vi "Grade IO Test.vi"(8 "Data Map":T5(array[cluster]) {"OPC UA Data Type" items=["Boolean"=1, "SByte"=2, "Byte"=3, "Int16"=4, "UInt16"=5, "Int32"=6, "UInt32"=7, "Int64"=8, "UInt64"=9, "Float"=10, "Double"=11, "String"=12, "DateTime"=13, "ByteString"=15, "Array of Boolean"=101, "Array of SByte"=102, "Array of Byte"=103, "Array of Int16"=104, "Array of UInt16"=105, "Array of Int32"=106, "Array of UInt32"=107, "Array of Int64"=108, "Array of UInt64"=109, "Array of Float"=110, "Array of Double"=111, "Array of String"=112, "Array of DateTime"=113, "Array of ByteString"=115]}, 9 "Server Data":T1(array[cluster]), 10 "data table in":T2) -> (2 "Pass?":bool[](array[boolean]))   [LabVIEW 2014, in "OPC UA Client Tests.lvlib"]
doc: "Checks to see that the Server Data (data written using OPC UA Server API) matches what is in the module's data table. Input map is used to map data table items to server data items."
uses:
  OPC UA Client Tests.lvlib
  <vilib>/NI/Tag Bus/tag/Data Type.ctl
  module/configuration/OPC UA Data Type.ctl
  <vilib>/NI/Tag Bus/table/data table.ctl
  <vilib>/NI/Tag Bus/table/data polymorphs/read one/read Boolean.vi
  <vilib>/NI/Tag Bus/table/data polymorphs/read one/read I8.vi
  <vilib>/NI/Tag Bus/table/data polymorphs/read one/read U8.vi
  <vilib>/NI/Tag Bus/table/data polymorphs/read one/read I16.vi
  <vilib>/NI/Tag Bus/table/data polymorphs/read one/read U16.vi
  <vilib>/NI/Tag Bus/table/data polymorphs/read one/read I32.vi
  <vilib>/NI/Tag Bus/table/data polymorphs/read one/read U32.vi
  <vilib>/NI/Tag Bus/table/data polymorphs/read one/read I64.vi
  <vilib>/NI/Tag Bus/table/data polymorphs/read one/read U64.vi
  <vilib>/NI/Tag Bus/table/data polymorphs/read one/read Single.vi
  <vilib>/NI/Tag Bus/table/data polymorphs/read one/read Double.vi
  <vilib>/NI/Tag Bus/table/data polymorphs/read one/read String.vi
  <vilib>/NI/Tag Bus/table/data polymorphs/read one/read Array of Boolean.vi
  <vilib>/NI/Tag Bus/table/data polymorphs/read one/read Array of I8.vi
  <vilib>/NI/Tag Bus/table/data polymorphs/read one/read Array of U8.vi
  <vilib>/NI/Tag Bus/table/data polymorphs/read one/read Array of I16.vi
  <vilib>/NI/Tag Bus/table/data polymorphs/read one/read Array of U16.vi
  <vilib>/NI/Tag Bus/table/data polymorphs/read one/read Array of I32.vi
  <vilib>/NI/Tag Bus/table/data polymorphs/read one/read Array of U32.vi
  <vilib>/NI/Tag Bus/table/data polymorphs/read one/read Array of I64.vi
  <vilib>/NI/Tag Bus/table/data polymorphs/read one/read Array of U64.vi
  <vilib>/NI/Tag Bus/table/data polymorphs/read one/read Array of Single.vi
  <vilib>/NI/Tag Bus/table/data polymorphs/read one/read Array of Double.vi
  <vilib>/NI/Tag Bus/table/data polymorphs/read one/read Array of String.vi
  <vilib>/NI/Tag Bus/table/data table.lvlib
  module/execution/OPC UA Client runtime.lvclass
  <vilib>/NI/Tag Bus/tag/tag descriptor.lvclass
  module/configuration/OPC UA Client configuration.lvclass
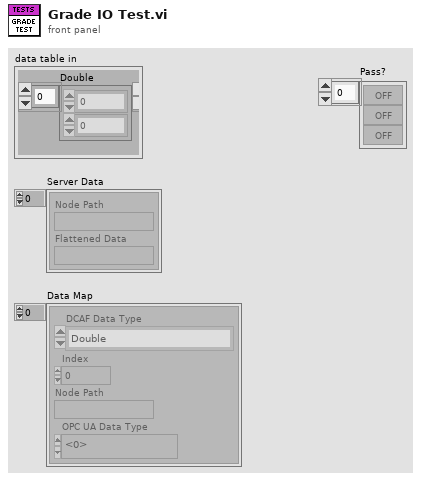
[diagram p1: front panel]
types:
  T1 = cluster{"Node Path":string, "Flattened Data":string}[]
  T2 = typedef "tag bus.lvlib/data table.lvlib/data table.ctl" = cluster{"Double":dbl[], "Single":sgl[], "I64":i64[], "I32":i32[], "I16":i16[], "I8":i8[], "U64":u64[], "U32":u32[], "U16":u16[], "U8":u8[], "Boolean":bool[], "String":string[], "Array of Double":cluster{"DBL Array":dbl[]}[], "Array of Single":cluster{"SGL Array":sgl[]}[], "Array of I64":cluster{"I64 Array":i64[]}[], "Array of I32":cluster{"I32 Array":i32[]}[], "Array of I16":cluster{"I16 Array":i16[]}[], "Array of I8":cluster{"I8 Array":i8[]}[], "Array of U64":cluster{"U64 Array":u64[]}[], "Array of U32":cluster{"U32 Array":u32[]}[], "Array of U16":cluster{"U16 Array":u16[]}[], "Array of U8":cluster{"U8 Array":u8[]}[], "Array of Boolean":cluster{"Boolean Array":bool[]}[], "Array of String":cluster{"String Array":string[]}[]}
  T3 = typedef "tag bus.lvlib/tag descriptor.lvclass/Data Type.ctl" = enum16{"Double", "Single", "I64", "I32", "I16", "I8", "U64", "U32", "U16", "U8", "Boolean", "String", "Array of Double", "Array of Single", "Array of I64", "Array of I32", "Array of I16", "Array of I8", "Array of U64", "Array of U32", "Array of U16", "Array of U8", "Array of Boolean", "Array of String"}
  T4 = typedef "OPC UA Client configuration.lvclass/OPC UA Data Type.ctl" = u16
  T5 = cluster{"DCAF Data Type":T3, "Index":i32, "Node Path":string, "OPC UA Data Type":T4}[]
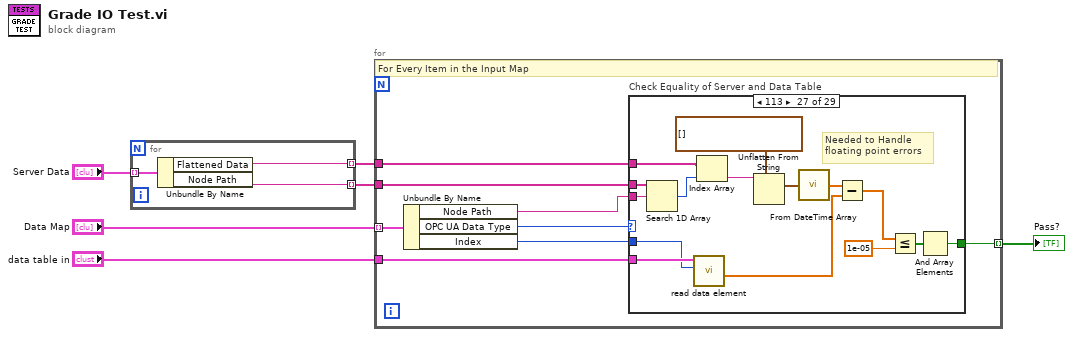
[diagram p0: block diagram]
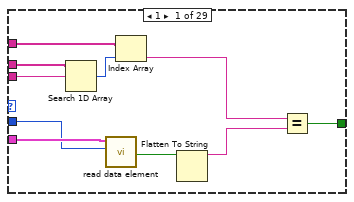
[diagram p2: hidden frame]
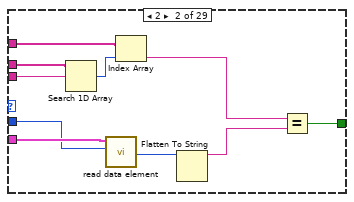
[diagram p3: hidden frame]
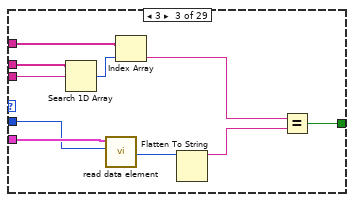
[diagram p4: hidden frame]
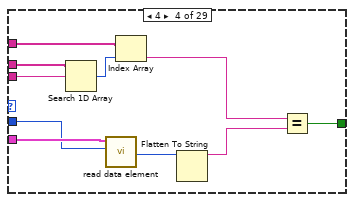
[diagram p5: hidden frame]
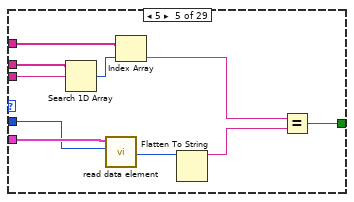
[diagram p6: hidden frame]
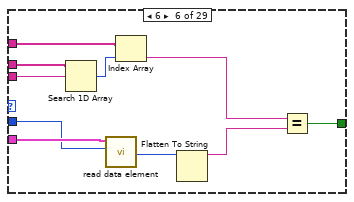
[diagram p7: hidden frame]
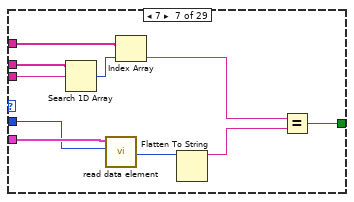
[diagram p8: hidden frame]
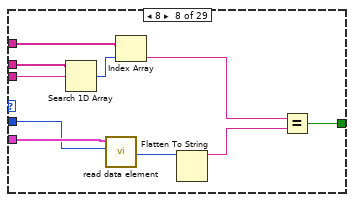
[diagram p9: hidden frame]
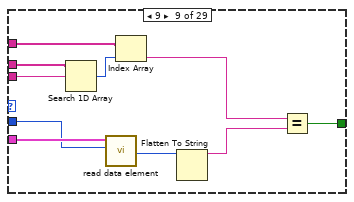
[diagram p10: hidden frame]
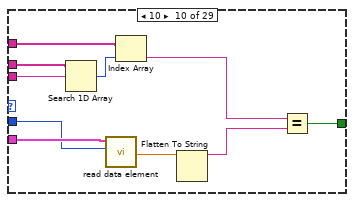
[diagram p11: hidden frame]
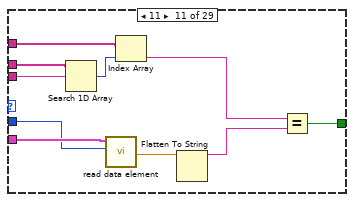
[diagram p12: hidden frame]
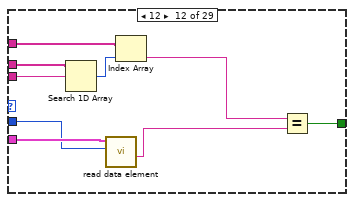
[diagram p13: hidden frame]
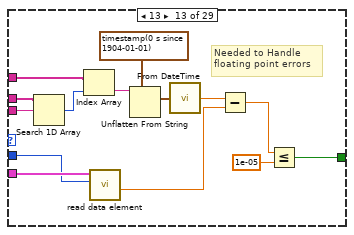
[diagram p14: hidden frame]
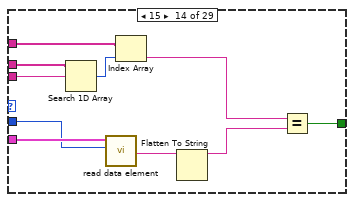
[diagram p15: hidden frame]
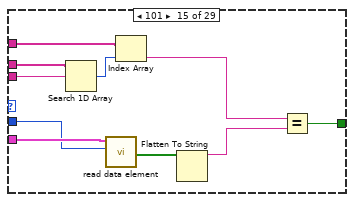
[diagram p16: hidden frame]
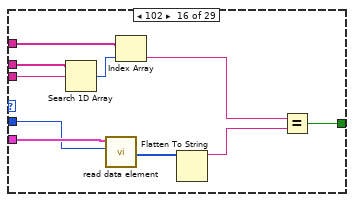
[diagram p17: hidden frame]
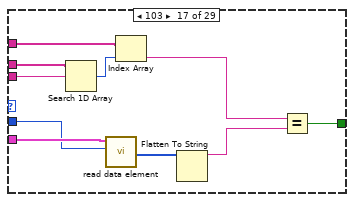
[diagram p18: hidden frame]
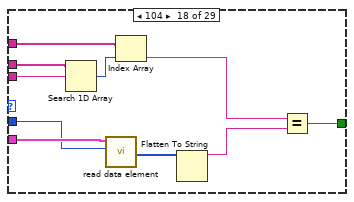
[diagram p19: hidden frame]
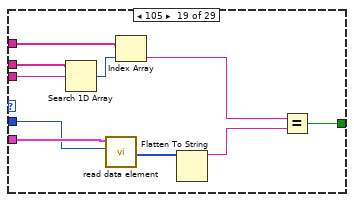
[diagram p20: hidden frame]
diagram:
  n1 = for {
    tunnel: "Server Data" -> [w9] mode=indexing
    tunnel: [w8] -> w3 mode=indexing
    tunnel: [w7] -> w2 mode=indexing
    n2 = Unbundle By Name(w9) -> ("Flattened Data"=w8:string, "Node Path"=w7:string)
  }
  n3 = for {
    tunnel: "Data Map" -> [w17] mode=indexing
    tunnel: "data table in" -> [w16]
    tunnel: w3 -> [w12]
    tunnel: w2 -> [w11]
    tunnel: [w10] -> w1 mode=indexing
    # "For Every Item in the Input Map"
    n4 = Unbundle By Name(w17) -> ("Node Path"=w14:string, "OPC UA Data Type"=w15:T4, "Index"=w13:i32)
    n5 = case "Check Equality of Server and Data Table" shown="113" w15 {
      tunnel: w16 -> [w23 w33 w43 w53 w63 w73 w83 w93 w103 w113 w123 w133 w149 w156 w166 w176 w186 w196 w206 w216 w226 w236 w246 w256 w266 w276 w294 w301 _]
      tunnel: w14 -> [w22 w32 w42 w52 w62 w72 w82 w92 w102 w112 w122 w132 w148 w155 w165 w175 w185 w195 w205 w215 w225 w235 w245 w255 w265 w275 w293 w300 _]
      tunnel: w13 -> [w21 w31 w41 w51 w61 w71 w81 w91 w101 w111 w121 w131 w147 w154 w164 w174 w184 w194 w204 w214 w224 w234 w244 w254 w264 w274 w292 w299 _]
      tunnel: w12 -> [w20 w30 w40 w50 w60 w70 w80 w90 w100 w110 w120 w130 w146 w153 w163 w173 w183 w193 w203 w213 w223 w233 w243 w253 w263 w273 w291 w298 _]
      tunnel: w11 -> [w19 w29 w39 w49 w59 w69 w79 w89 w99 w109 w119 w129 w145 w152 w162 w172 w182 w192 w202 w212 w222 w232 w242 w252 w262 w272 w290 w297 _]
      tunnel: [w18 w28 w38 w48 w58 w68 w78 w88 w98 w108 w118 w128 w138 w151 w161 w171 w181 w191 w201 w211 w221 w231 w241 w251 w261 w271 w281 w296 FALSE] -> w10
      frame 1 {
        n6 = Search 1D Array(1D array=w19, element=w22) -> (index of element=w25:i32)  [unwired: 1 in]
        n7 = call-poly <vilib>:"read data element.vi"("index"=w21, "data table in"=w23) -> ("value"=w24:bool)  [unwired: 8 in, 1 out]
        n8 = Index Array(array=w20, index=w25) -> (element=w27:string)
        n9 = Flatten To String(anything=w24) -> (data string=w26:string)  [unwired: 3 in, 2 out]
        n10 = Equal?(x=w27, y=w26) -> (x = y?=w18:bool)
      }
      frame 2 {
        n11 = Search 1D Array(1D array=w29, element=w32) -> (index of element=w35:i32)  [unwired: 1 in]
        n12 = call-poly <vilib>:"read data element.vi"("index"=w31, "data table in"=w33) -> ("value"=w34:i8)  [unwired: 8 in, 1 out]
        n13 = Index Array(array=w30, index=w35) -> (element=w37:string)
        n14 = Flatten To String(anything=w34) -> (data string=w36:string)  [unwired: 3 in, 2 out]
        n15 = Equal?(x=w37, y=w36) -> (x = y?=w28:bool)
      }
      frame 3 {
        n16 = Search 1D Array(1D array=w39, element=w42) -> (index of element=w45:i32)  [unwired: 1 in]
        n17 = call-poly <vilib>:"read data element.vi"("index"=w41, "data table in"=w43) -> ("value"=w44:u8)  [unwired: 8 in, 1 out]
        n18 = Index Array(array=w40, index=w45) -> (element=w47:string)
        n19 = Flatten To String(anything=w44) -> (data string=w46:string)  [unwired: 3 in, 2 out]
        n20 = Equal?(x=w47, y=w46) -> (x = y?=w38:bool)
      }
      frame 4 {
        n21 = Search 1D Array(1D array=w49, element=w52) -> (index of element=w55:i32)  [unwired: 1 in]
        n22 = call-poly <vilib>:"read data element.vi"("index"=w51, "data table in"=w53) -> ("value"=w54:i16)  [unwired: 8 in, 1 out]
        n23 = Index Array(array=w50, index=w55) -> (element=w57:string)
        n24 = Flatten To String(anything=w54) -> (data string=w56:string)  [unwired: 3 in, 2 out]
        n25 = Equal?(x=w57, y=w56) -> (x = y?=w48:bool)
      }
      frame 5 {
        n26 = Search 1D Array(1D array=w59, element=w62) -> (index of element=w65:i32)  [unwired: 1 in]
        n27 = call-poly <vilib>:"read data element.vi"("index"=w61, "data table in"=w63) -> ("value"=w64:u16)  [unwired: 8 in, 1 out]
        n28 = Index Array(array=w60, index=w65) -> (element=w67:string)
        n29 = Flatten To String(anything=w64) -> (data string=w66:string)  [unwired: 3 in, 2 out]
        n30 = Equal?(x=w67, y=w66) -> (x = y?=w58:bool)
      }
      frame 6 {
        n31 = Search 1D Array(1D array=w69, element=w72) -> (index of element=w75:i32)  [unwired: 1 in]
        n32 = call-poly <vilib>:"read data element.vi"("index"=w71, "data table in"=w73) -> ("value"=w74:i32)  [unwired: 8 in, 1 out]
        n33 = Index Array(array=w70, index=w75) -> (element=w77:string)
        n34 = Flatten To String(anything=w74) -> (data string=w76:string)  [unwired: 3 in, 2 out]
        n35 = Equal?(x=w77, y=w76) -> (x = y?=w68:bool)
      }
      frame 7 {
        n36 = Search 1D Array(1D array=w79, element=w82) -> (index of element=w85:i32)  [unwired: 1 in]
        n37 = call-poly <vilib>:"read data element.vi"("index"=w81, "data table in"=w83) -> ("value"=w84:u32)  [unwired: 8 in, 1 out]
        n38 = Index Array(array=w80, index=w85) -> (element=w87:string)
        n39 = Flatten To String(anything=w84) -> (data string=w86:string)  [unwired: 3 in, 2 out]
        n40 = Equal?(x=w87, y=w86) -> (x = y?=w78:bool)
      }
      frame 8 {
        n41 = Search 1D Array(1D array=w89, element=w92) -> (index of element=w95:i32)  [unwired: 1 in]
        n42 = call-poly <vilib>:"read data element.vi"("index"=w91, "data table in"=w93) -> ("value"=w94:i64)  [unwired: 8 in, 1 out]
        n43 = Index Array(array=w90, index=w95) -> (element=w97:string)
        n44 = Flatten To String(anything=w94) -> (data string=w96:string)  [unwired: 3 in, 2 out]
        n45 = Equal?(x=w97, y=w96) -> (x = y?=w88:bool)
      }
      frame 9 {
        n46 = Search 1D Array(1D array=w99, element=w102) -> (index of element=w105:i32)  [unwired: 1 in]
        n47 = call-poly <vilib>:"read data element.vi"("index"=w101, "data table in"=w103) -> ("value"=w104:u64)  [unwired: 8 in, 1 out]
        n48 = Index Array(array=w100, index=w105) -> (element=w107:string)
        n49 = Flatten To String(anything=w104) -> (data string=w106:string)  [unwired: 3 in, 2 out]
        n50 = Equal?(x=w107, y=w106) -> (x = y?=w98:bool)
      }
      frame 10 {
        n51 = Search 1D Array(1D array=w109, element=w112) -> (index of element=w115:i32)  [unwired: 1 in]
        n52 = call-poly <vilib>:"read data element.vi"("index"=w111, "data table in"=w113) -> ("value"=w114:sgl)  [unwired: 8 in, 1 out]
        n53 = Index Array(array=w110, index=w115) -> (element=w117:string)
        n54 = Flatten To String(anything=w114) -> (data string=w116:string)  [unwired: 3 in, 2 out]
        n55 = Equal?(x=w117, y=w116) -> (x = y?=w108:bool)
      }
      frame 11 {
        n56 = Search 1D Array(1D array=w119, element=w122) -> (index of element=w125:i32)  [unwired: 1 in]
        n57 = call-poly <vilib>:"read data element.vi"("index"=w121, "data table in"=w123) -> ("value"=w124:dbl)  [unwired: 8 in, 1 out]
        n58 = Index Array(array=w120, index=w125) -> (element=w127:string)
        n59 = Flatten To String(anything=w124) -> (data string=w126:string)  [unwired: 3 in, 2 out]
        n60 = Equal?(x=w127, y=w126) -> (x = y?=w118:bool)
      }
      frame 12 {
        n61 = Search 1D Array(1D array=w129, element=w132) -> (index of element=w135:i32)  [unwired: 1 in]
        n62 = call-poly <vilib>:"read data element.vi"("index"=w131, "data table in"=w133) -> ("value"=w134:string)  [unwired: 8 in, 1 out]
        n63 = Index Array(array=w130, index=w135) -> (element=w136:string)
        n64 = Equal?(x=w136, y=w134) -> (x = y?=w128:bool)
      }
      frame 13 {
        # "Needed to Handle\nfloating point errors"
        n65 = Search 1D Array(1D array=w145, element=w148) -> (index of element=w150:i32)  [unwired: 1 in]
        n66 = Index Array(array=w146, index=w150) -> (element=w144:string)
        n67 = call-poly <vilib>:"read data element.vi"("index"=w147, "data table in"=w149) -> ("value"=w140:dbl)  [unwired: 8 in, 1 out]
        n68 = Unflatten From String(type=timestamp(0 s since 1904-01-01) ("value"), binary string=w144) -> (value=w142:timestamp)  [unwired: 3 in, 2 out]
        n69 = call "From DateTime.vi"("DateTime"=w142) -> ("Formatted DateTime"=w141:dbl)
        n70 = Subtract(x=w141, y=w140) -> (x-y=w139:dbl)
        n71 = Less Or Equal?(x=w139, y=1e-05) -> (x <= y?=w138:bool)
      }
      frame 15 {
        n72 = Search 1D Array(1D array=w152, element=w155) -> (index of element=w158:i32)  [unwired: 1 in]
        n73 = call-poly <vilib>:"read data element.vi"("index"=w154, "data table in"=w156) -> ("value"=w157:string)  [unwired: 8 in, 1 out]
        n74 = Index Array(array=w153, index=w158) -> (element=w160:string)
        n75 = Flatten To String(anything=w157) -> (data string=w159:string)  [unwired: 3 in, 2 out]
        n76 = Equal?(x=w160, y=w159) -> (x = y?=w151:bool)
      }
      frame 101 {
        n77 = Search 1D Array(1D array=w162, element=w165) -> (index of element=w168:i32)  [unwired: 1 in]
        n78 = call-poly <vilib>:"read data element.vi"("index"=w164, "data table in"=w166) -> ("value"=w167:bool[])  [unwired: 8 in, 1 out]
        n79 = Index Array(array=w163, index=w168) -> (element=w170:string)
        n80 = Flatten To String(anything=w167) -> (data string=w169:string)  [unwired: 3 in, 2 out]
        n81 = Equal?(x=w170, y=w169) -> (x = y?=w161:bool)
      }
      frame 102 {
        n82 = Search 1D Array(1D array=w172, element=w175) -> (index of element=w178:i32)  [unwired: 1 in]
        n83 = call-poly <vilib>:"read data element.vi"("index"=w174, "data table in"=w176) -> ("value"=w177:i8[])  [unwired: 8 in, 1 out]
        n84 = Index Array(array=w173, index=w178) -> (element=w180:string)
        n85 = Flatten To String(anything=w177) -> (data string=w179:string)  [unwired: 3 in, 2 out]
        n86 = Equal?(x=w180, y=w179) -> (x = y?=w171:bool)
      }
      frame 103 {
        n87 = Search 1D Array(1D array=w182, element=w185) -> (index of element=w188:i32)  [unwired: 1 in]
        n88 = call-poly <vilib>:"read data element.vi"("index"=w184, "data table in"=w186) -> ("value"=w187:u8[])  [unwired: 8 in, 1 out]
        n89 = Index Array(array=w183, index=w188) -> (element=w190:string)
        n90 = Flatten To String(anything=w187) -> (data string=w189:string)  [unwired: 3 in, 2 out]
        n91 = Equal?(x=w190, y=w189) -> (x = y?=w181:bool)
      }
      frame 104 {
        n92 = Search 1D Array(1D array=w192, element=w195) -> (index of element=w198:i32)  [unwired: 1 in]
        n93 = call-poly <vilib>:"read data element.vi"("index"=w194, "data table in"=w196) -> ("value"=w197:i16[])  [unwired: 8 in, 1 out]
        n94 = Index Array(array=w193, index=w198) -> (element=w200:string)
        n95 = Flatten To String(anything=w197) -> (data string=w199:string)  [unwired: 3 in, 2 out]
        n96 = Equal?(x=w200, y=w199) -> (x = y?=w191:bool)
      }
      frame 105 {
        n97 = Search 1D Array(1D array=w202, element=w205) -> (index of element=w208:i32)  [unwired: 1 in]
        n98 = call-poly <vilib>:"read data element.vi"("index"=w204, "data table in"=w206) -> ("value"=w207:u16[])  [unwired: 8 in, 1 out]
        n99 = Index Array(array=w203, index=w208) -> (element=w210:string)
        n100 = Flatten To String(anything=w207) -> (data string=w209:string)  [unwired: 3 in, 2 out]
        n101 = Equal?(x=w210, y=w209) -> (x = y?=w201:bool)
      }
      frame 106 {
        n102 = Search 1D Array(1D array=w212, element=w215) -> (index of element=w218:i32)  [unwired: 1 in]
        n103 = call-poly <vilib>:"read data element.vi"("index"=w214, "data table in"=w216) -> ("value"=w217:i32[])  [unwired: 8 in, 1 out]
        n104 = Index Array(array=w213, index=w218) -> (element=w220:string)
        n105 = Flatten To String(anything=w217) -> (data string=w219:string)  [unwired: 3 in, 2 out]
        n106 = Equal?(x=w220, y=w219) -> (x = y?=w211:bool)
      }
      frame 107 {
        n107 = Search 1D Array(1D array=w222, element=w225) -> (index of element=w228:i32)  [unwired: 1 in]
        n108 = call-poly <vilib>:"read data element.vi"("index"=w224, "data table in"=w226) -> ("value"=w227:u32[])  [unwired: 8 in, 1 out]
        n109 = Index Array(array=w223, index=w228) -> (element=w230:string)
        n110 = Flatten To String(anything=w227) -> (data string=w229:string)  [unwired: 3 in, 2 out]
        n111 = Equal?(x=w230, y=w229) -> (x = y?=w221:bool)
      }
      frame 108 {
        n112 = Search 1D Array(1D array=w232, element=w235) -> (index of element=w238:i32)  [unwired: 1 in]
        n113 = call-poly <vilib>:"read data element.vi"("index"=w234, "data table in"=w236) -> ("value"=w237:i64[])  [unwired: 8 in, 1 out]
        n114 = Index Array(array=w233, index=w238) -> (element=w240:string)
        n115 = Flatten To String(anything=w237) -> (data string=w239:string)  [unwired: 3 in, 2 out]
        n116 = Equal?(x=w240, y=w239) -> (x = y?=w231:bool)
      }
      frame 109 {
        n117 = Search 1D Array(1D array=w242, element=w245) -> (index of element=w248:i32)  [unwired: 1 in]
        n118 = call-poly <vilib>:"read data element.vi"("index"=w244, "data table in"=w246) -> ("value"=w247:u64[])  [unwired: 8 in, 1 out]
        n119 = Index Array(array=w243, index=w248) -> (element=w250:string)
        n120 = Flatten To String(anything=w247) -> (data string=w249:string)  [unwired: 3 in, 2 out]
        n121 = Equal?(x=w250, y=w249) -> (x = y?=w241:bool)
      }
      frame 110 {
        n122 = Search 1D Array(1D array=w252, element=w255) -> (index of element=w258:i32)  [unwired: 1 in]
        n123 = call-poly <vilib>:"read data element.vi"("index"=w254, "data table in"=w256) -> ("value"=w257:sgl[])  [unwired: 8 in, 1 out]
        n124 = Index Array(array=w253, index=w258) -> (element=w260:string)
        n125 = Flatten To String(anything=w257) -> (data string=w259:string)  [unwired: 3 in, 2 out]
        n126 = Equal?(x=w260, y=w259) -> (x = y?=w251:bool)
      }
      frame 111 {
        n127 = Search 1D Array(1D array=w262, element=w265) -> (index of element=w268:i32)  [unwired: 1 in]
        n128 = call-poly <vilib>:"read data element.vi"("index"=w264, "data table in"=w266) -> ("value"=w267:dbl[])  [unwired: 8 in, 1 out]
        n129 = Index Array(array=w263, index=w268) -> (element=w270:string)
        n130 = Flatten To String(anything=w267) -> (data string=w269:string)  [unwired: 3 in, 2 out]
        n131 = Equal?(x=w270, y=w269) -> (x = y?=w261:bool)
      }
      frame 112 {
        n132 = Search 1D Array(1D array=w272, element=w275) -> (index of element=w278:i32)  [unwired: 1 in]
        n133 = call-poly <vilib>:"read data element.vi"("index"=w274, "data table in"=w276) -> ("value"=w277:string[])  [unwired: 8 in, 1 out]
        n134 = Index Array(array=w273, index=w278) -> (element=w280:string)
        n135 = Flatten To String(anything=w277) -> (data string=w279:string)  [unwired: 3 in, 2 out]
        n136 = Equal?(x=w280, y=w279) -> (x = y?=w271:bool)
      }
      frame 113 {
        # "Needed to Handle\nfloating point errors"
        n137 = Search 1D Array(1D array=w290, element=w293) -> (index of element=w295:i32)  [unwired: 1 in]
        n138 = call-poly <vilib>:"read data element.vi"("index"=w292, "data table in"=w294) -> ("value"=w288:dbl[])  [unwired: 8 in, 1 out]
        n139 = Index Array(array=w291, index=w295) -> (element=w289:string)
        n140 = Unflatten From String(type=timestamp[] [], binary string=w289) -> (value=w286:timestamp[])  [unwired: 3 in, 2 out]
        n141 = call "From DateTime Array.vi"("DateTime Array"=w286) -> ("Formatted DateTime Array"=w285:dbl[])
        n142 = Subtract(x=w285, y=w288) -> (x-y=w284:dbl[])
        n143 = Less Or Equal?(x=w284, y=1e-05) -> (x <= y?=w282:bool[])
        n144 = And Array Elements(Boolean array=w282) -> (logical AND=w281:bool)
      }
      frame 115 {
        n145 = Search 1D Array(1D array=w297, element=w300) -> (index of element=w303:i32)  [unwired: 1 in]
        n146 = call-poly <vilib>:"read data element.vi"("index"=w299, "data table in"=w301) -> ("value"=w302:string)  [unwired: 8 in, 1 out]
        n147 = Index Array(array=w298, index=w303) -> (element=w305:string)
        n148 = Flatten To String(anything=w302) -> (data string=w304:string)  [unwired: 3 in, 2 out]
        n149 = Equal?(x=w305, y=w304) -> (x = y?=w296:bool)
      }
      frame 0, Default {
      }
    }
  }
  "Pass?" <- w1
